vi "Lidar_data_to_array.vi"(8 "error in":errorcluster, 10 "Data":cluster{"Angle":dbl, dbl}[](array[cluster])=[{"Angle"=0.21875, 4216.25}, {"Angle"=1.453125, 4215.0}, {"Angle"=2.703125, 4202.75}, {"Angle"=3.921875, 4227.5}, {"Angle"=8.921875, 4154.5}, {"Angle"=10.15625, 4172.25}, {"Angle"=11.421875, 4185.25}, {"Angle"=12.65625, 4214.75}, {"Angle"=13.890625, 4259.75}, {"Angle"=15.140625, 4138.75}, {"Angle"=26.734375, 1918.75}, {"Angle"=28.03125, 1787.5}, {"Angle"=29.296875, 1698.75}, {"Angle"=30.609375, 1615.5}, {"Angle"=31.921875, 1550.0}, {"Angle"=33.171875, 1481.0}, {"Angle"=34.4375, 1424.5}, {"Angle"=35.890625, 1366.5}, {"Angle"=37.109375, 1322.75}, {"Angle"=38.46875, 1274.5}, {"Angle"=39.75, 1229.25}, {"Angle"=41.046875, 1186.75}, {"Angle"=42.28125, 1149.25}, {"Angle"=43.53125, 1118.5}, {"Angle"=45.46875, 738.25}, {"Angle"=46.828125, 686.75}, {"Angle"=48.25, 667.25}, {"Angle"=49.640625, 646.25}, {"Angle"=50.765625, 633.0}, {"Angle"=52.0, 625.5}, {"Angle"=53.28125, 619.5}, {"Angle"=54.5625, 618.5}, {"Angle"=55.890625, 616.25}, {"Angle"=57.203125, 610.0}, {"Angle"=58.3125, 609.5}, {"Angle"=59.71875, 608.25}, {"Angle"=60.921875, 622.5}, {"Angle"=62.0625, 628.25}, {"Angle"=63.328125, 641.0}, {"Angle"=64.4375, 665.25}, {"Angle"=65.6875, 672.5}, {"Angle"=66.828125, 679.5}, {"Angle"=68.15625, 693.25}, {"Angle"=69.28125, 705.75}, {"Angle"=70.484375, 720.25}, {"Angle"=71.75, 710.0}, {"Angle"=73.171875, 701.5}, {"Angle"=74.296875, 699.0}, {"Angle"=75.625, 690.0}, {"Angle"=76.78125, 683.0}, {"Angle"=78.1875, 678.25}, {"Angle"=79.46875, 673.75}, {"Angle"=80.734375, 671.0}, {"Angle"=81.9375, 666.5}, {"Angle"=83.15625, 663.5}, {"Angle"=84.46875, 660.75}, {"Angle"=85.703125, 657.0}, {"Angle"=87.015625, 652.25}, {"Angle"=88.0625, 651.0}, {"Angle"=89.46875, 645.5}, {"Angle"=90.59375, 644.5}, {"Angle"=91.890625, 644.25}, {"Angle"=93.125, 643.5}, {"Angle"=94.484375, 642.25}, {"Angle"=95.65625, 640.75}, {"Angle"=97.015625, 640.0}, {"Angle"=98.0625, 641.75}, {"Angle"=99.421875, 642.25}, {"Angle"=100.59375, 642.0}, {"Angle"=101.859375, 645.0}, {"Angle"=103.109375, 647.0}, {"Angle"=104.25, 650.25}, {"Angle"=105.640625, 653.0}, {"Angle"=106.78125, 658.0}, {"Angle"=108.140625, 660.25}, {"Angle"=109.140625, 662.5}, {"Angle"=110.40625, 665.25}, {"Angle"=111.65625, 670.0}, {"Angle"=112.828125, 676.5}, {"Angle"=114.03125, 701.25}, {"Angle"=115.359375, 704.25}, {"Angle"=116.625, 710.25}, {"Angle"=117.828125, 717.0}, {"Angle"=119.046875, 722.5}, {"Angle"=120.21875, 727.25}, {"Angle"=121.40625, 737.0}, {"Angle"=122.671875, 745.75}, {"Angle"=123.8125, 756.25}, {"Angle"=125.03125, 764.0}, {"Angle"=126.328125, 774.0}, {"Angle"=127.5, 780.0}, {"Angle"=128.75, 792.0}, {"Angle"=129.96875, 807.75}, {"Angle"=131.25, 816.75}, {"Angle"=132.5, 830.0}, {"Angle"=133.703125, 847.25}, {"Angle"=134.90625, 862.75}, {"Angle"=136.015625, 877.0}, {"Angle"=137.203125, 893.5}, {"Angle"=138.53125, 911.75}, {"Angle"=139.75, 931.5}, {"Angle"=140.890625, 953.75}, {"Angle"=142.15625, 970.75}, {"Angle"=143.28125, 996.5}, {"Angle"=147.109375, 977.75}, {"Angle"=148.375, 956.5}, {"Angle"=149.625, 941.5}, {"Angle"=150.84375, 927.25}, {"Angle"=152.109375, 913.5}, {"Angle"=153.375, 896.75}, {"Angle"=154.65625, 883.5}, {"Angle"=156.046875, 873.5}, {"Angle"=157.3125, 862.75}, {"Angle"=158.578125, 852.5}, {"Angle"=159.828125, 842.75}, {"Angle"=161.03125, 835.75}, {"Angle"=162.28125, 826.75}, {"Angle"=163.5, 819.0}, {"Angle"=164.765625, 810.75}, {"Angle"=166.109375, 803.75}, {"Angle"=167.421875, 795.5}, {"Angle"=168.53125, 789.75}, {"Angle"=169.921875, 781.75}, {"Angle"=171.171875, 778.0}, {"Angle"=172.390625, 776.25}, {"Angle"=173.703125, 770.25}, {"Angle"=174.9375, 767.0}, {"Angle"=176.125, 764.0}, {"Angle"=177.390625, 762.0}, {"Angle"=178.609375, 762.75}, {"Angle"=179.828125, 757.75}, {"Angle"=181.09375, 756.0}, {"Angle"=182.4375, 753.75}, {"Angle"=183.6875, 750.75}, {"Angle"=184.84375, 751.75}, {"Angle"=186.0625, 751.25}, {"Angle"=187.40625, 753.25}, {"Angle"=188.578125, 752.0}, {"Angle"=189.859375, 753.25}, {"Angle"=191.125, 757.5}, {"Angle"=192.296875, 758.25}, {"Angle"=193.59375, 758.5}, {"Angle"=194.78125, 763.75}, {"Angle"=196.0625, 767.75}, {"Angle"=197.296875, 768.0}, {"Angle"=198.5, 771.25}, {"Angle"=199.71875, 775.0}, {"Angle"=201.0625, 779.75}, {"Angle"=202.15625, 785.5}, {"Angle"=203.46875, 791.5}, {"Angle"=204.6875, 795.75}, {"Angle"=205.890625, 804.25}, {"Angle"=207.25, 810.75}, {"Angle"=208.40625, 818.0}, {"Angle"=209.640625, 823.25}, {"Angle"=210.890625, 834.75}, {"Angle"=212.15625, 843.5}, {"Angle"=213.375, 849.25}, {"Angle"=214.578125, 863.0}, {"Angle"=215.71875, 869.75}, {"Angle"=216.984375, 884.0}, {"Angle"=218.25, 895.5}, {"Angle"=219.5, 905.75}, {"Angle"=221.484375, 634.0}, {"Angle"=222.84375, 592.25}, {"Angle"=224.171875, 580.0}, {"Angle"=225.3125, 575.25}, {"Angle"=226.765625, 560.25}, {"Angle"=228.0, 548.25}, {"Angle"=229.3125, 541.0}, {"Angle"=230.4375, 538.0}, {"Angle"=234.296875, 541.0}, {"Angle"=235.4375, 550.0}, {"Angle"=236.828125, 550.0}, {"Angle"=237.9375, 564.5}, {"Angle"=243.796875, 1442.5}, {"Angle"=245.03125, 1497.25}, {"Angle"=246.1875, 1545.75}, {"Angle"=247.421875, 1604.25}, {"Angle"=248.640625, 1664.75}, {"Angle"=249.875, 1738.5}, {"Angle"=251.0625, 1806.25}, {"Angle"=252.25, 1897.0}, {"Angle"=253.46875, 1989.75}, {"Angle"=254.65625, 2093.75}, {"Angle"=255.859375, 2232.25}, {"Angle"=260.921875, 2091.25}, {"Angle"=263.40625, 2057.0}, {"Angle"=265.75, 2575.75}, {"Angle"=266.984375, 2633.25}, {"Angle"=268.234375, 2660.5}, {"Angle"=269.453125, 2648.75}, {"Angle"=270.734375, 2645.5}, {"Angle"=271.953125, 2634.5}, {"Angle"=273.171875, 2895.75}, {"Angle"=274.421875, 2922.25}, {"Angle"=275.578125, 2911.75}, {"Angle"=276.859375, 2751.0}, {"Angle"=278.125, 2639.75}, {"Angle"=279.359375, 2585.25}, {"Angle"=280.53125, 3051.25}, {"Angle"=281.78125, 3052.0}, {"Angle"=283.0, 3092.0}, {"Angle"=284.234375, 3066.5}, {"Angle"=285.484375, 3097.75}, {"Angle"=286.71875, 3103.0}, {"Angle"=287.96875, 3120.25}, {"Angle"=289.203125, 3137.75}, {"Angle"=290.421875, 3153.0}, {"Angle"=291.703125, 3161.25}, {"Angle"=292.921875, 3176.5}, {"Angle"=294.171875, 3198.5}, {"Angle"=295.390625, 3220.25}, {"Angle"=296.671875, 3060.5}, {"Angle"=297.953125, 2774.25}, {"Angle"=299.3125, 2809.0}, {"Angle"=300.578125, 2770.0}, {"Angle"=301.71875, 3362.75}, {"Angle"=303.078125, 2738.75}, {"Angle"=304.28125, 2945.5}, {"Angle"=305.546875, 2903.25}, {"Angle"=333.984375, 4913.5}, {"Angle"=335.21875, 4815.0}, {"Angle"=336.484375, 4728.5}, {"Angle"=337.71875, 4697.0}, {"Angle"=338.984375, 4677.5}, {"Angle"=340.234375, 4611.5}, {"Angle"=341.484375, 4570.25}, {"Angle"=342.734375, 4523.5}, {"Angle"=343.96875, 4483.75}, {"Angle"=345.234375, 4456.75}, {"Angle"=346.453125, 4444.0}, {"Angle"=347.6875, 4390.75}, {"Angle"=348.9375, 4382.0}, {"Angle"=350.171875, 4370.25}, {"Angle"=351.421875, 4200.0}, {"Angle"=352.765625, 4116.5}, {"Angle"=354.0, 4161.0}, {"Angle"=355.234375, 4281.75}, {"Angle"=356.46875, 4281.75}, {"Angle"=357.71875, 4247.75}, {"Angle"=358.96875, 4237.25}]) -> (0 "error out":errorcluster, 2 "Tableau lidar formaté":dbl[][](array[numeric])=[[0.0, 1.0, 2.0, 3.0, 4.0, 5.0, 6.0, 7.0, 8.0, 9.0, 10.0, 11.0, 12.0, 13.0, 14.0, 15.0, 16.0, 17.0, 18.0, 19.0, 20.0, 21.0, 22.0, 23.0, 24.0, 25.0, 26.0, 27.0, 28.0, 29.0, 30.0, 31.0, 32.0, 33.0, 34.0, 35.0], [20.0, 15.0, 30.0, 31.0, 42.0, 50.0, 51.0, 60.0, 20.0, 15.0, 30.0, 31.0, 42.0, 50.0, 51.0, 60.0, 20.0, 15.0, 30.0, 31.0, 42.0, 50.0, 51.0, 60.0, 20.0, 15.0, 30.0, 31.0, 42.0, 50.0, 51.0, 60.0, 20.0, 15.0, 30.0, 31.0], [0.0, 0.0, 0.0, 0.0, 0.0, 0.0, 0.0, 0.0, 0.0, 0.0, 0.0, 0.0, 0.0, 0.0, 0.0, 0.0, 0.0, 0.0, 0.0, 0.0, 0.0, 0.0, 0.0, 0.0, 0.0, 0.0, 0.0, 0.0, 0.0, 0.0, 0.0, 0.0, 0.0, 0.0, 0.0, 0.0]])   [LabVIEW 2018]
panel:
  out "Angle arrondi":dbl
  out "Angle":dbl
  out "Tableau lidar Init":dbl[][](array[numeric])
  out "Data array":dbl[](array[numeric])
  out "Data cluster":cluster{"Angle":dbl, dbl}
  # "Face Avant"
  # "Debug"
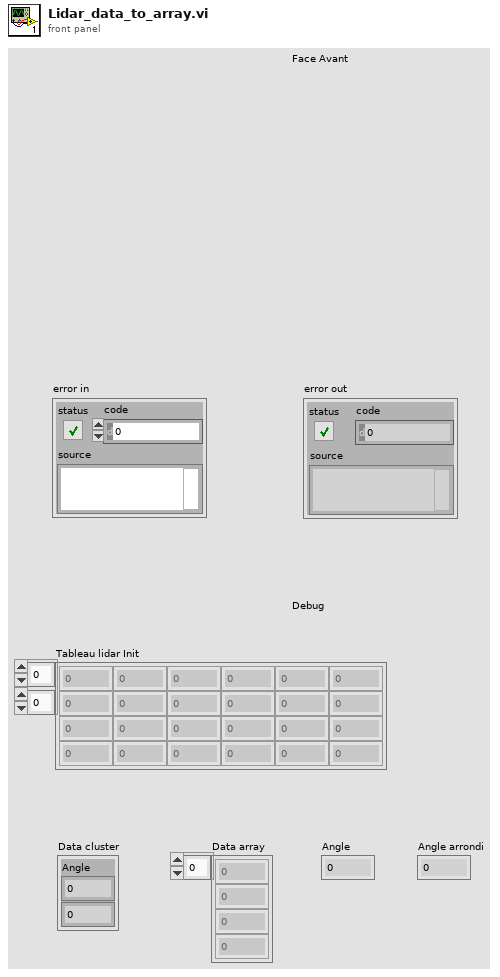
[diagram p1: front panel]
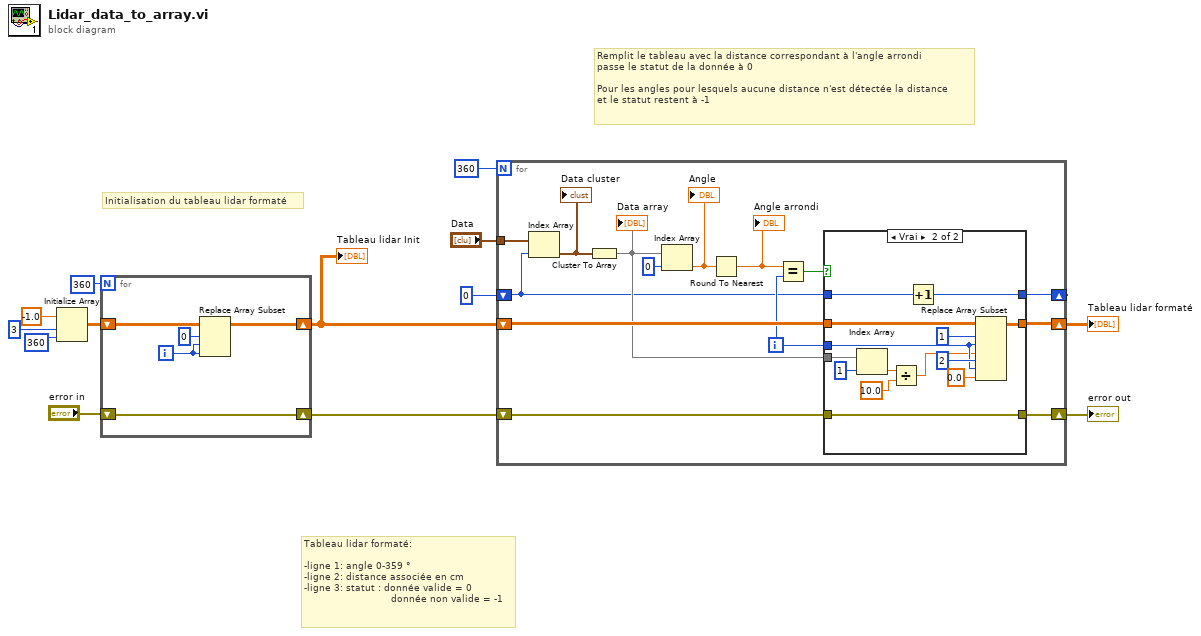
[diagram p0: block diagram]
diagram:
  # "Tableau lidar formaté:\n\n-ligne 1: angle 0-359 °\n-ligne 2: distance associée en cm\n-ligne 3: statut : donnée valide = 0\n                             donnée non valide = -1"
  # "Remplit le tableau avec la distance correspondant à l'angle arrondi\npasse le statut de la donnée à 0\n\nPour les angles pour lesquels aucune distance n'est détectée la distance\net le statut restent à -1"
  # "Initialisation du tableau lidar formaté"
  n1 = Initialize Array(-1.0 ("element"), 3 ("dimension size"), 360 ("dimension size")) -> (w7:dbl[][])
  n2 = for {
    N: 360 -> [_]
    shift-right: [w16] -> w6
    shift-left: w7 -> [w18]
    shift-right: [w14] -> w2
    shift-left: "error in" -> [w14]
    i -> [w15]
    n3 = Replace Array Subset(array=w18, new element=w15, index (row)=0 ("index"), index (col)=w15) -> (w16:dbl[][])
  }
  "Tableau lidar Init" <- w6
  n4 = for {
    N: 360 -> [_]
    shift-right: [w25] -> w9
    shift-left: w6 -> [w26]
    tunnel: "Data" -> [w31]
    shift-right: [w21] -> _
    shift-left: 0 -> [w22]
    shift-right: [w20] -> w1
    shift-left: w2 -> [w19]
    i -> [w24]
    n5 = Index Array(array=w31, index=w22) -> (element=w32:cluster{"Angle":dbl, dbl})
    "Data cluster" <- w32
    n6 = Cluster To Array(cluster=w32) -> (array=w23:dbl[])
    "Data array" <- w23
    n7 = Index Array(array=w23, index=0) -> (element=w29:dbl)
    "Angle" <- w29
    n8 = Round To Nearest(number=w29) -> (nearest integer value=w28:dbl)
    "Angle arrondi" <- w28
    n9 = Equal?(x=w28, y=w24) -> (x = y?=w27:bool)
    n10 = case shown="Vrai" w27 {
      tunnel: w26 -> [w35 w49]
      tunnel: [w35 w47] -> w25
      tunnel: w24 -> [_ w42]
      tunnel: w23 -> [_ w45]
      tunnel: w22 -> [w34 w41]
      tunnel: [w34 w40] -> w21
      tunnel: w19 -> [w33 w36]
      tunnel: [w33 w36] -> w20
      frame False {
      }
      frame True {
        n11 = Index Array(array=w45, index=1) -> (element=w38:dbl)
        n12 = Divide(x=w38, y=10.0) -> (x/y=w37:dbl)
        n13 = Increment(x=w41) -> (x+1=w40:i32)
        n14 = Replace Array Subset(array=w49, new element #1=w37, index (row) #1=1 ("index (row)"), index (col) #1=w42, new element #2=0.0 ("new element/subarray"), index (row) #2=2 ("index (row)"), index (col) #2=w42) -> (w47:dbl[][])
      }
    }
  }
  "Tableau lidar formaté" <- w9
  "error out" <- w1
